vi "TEST - LVOOP Return Class Name.vi"(8 "error in (no error)":errorcluster) -> (0 "error out":errorcluster, 2 "Pass":bool)   [LabVIEW 2020, in "test_openg_array.lvlib"]
uses:
  test_openg_array.lvlib
  LVOOP Data/Class 1/Class 1.lvclass
  source/library/openg_variant.lvlib
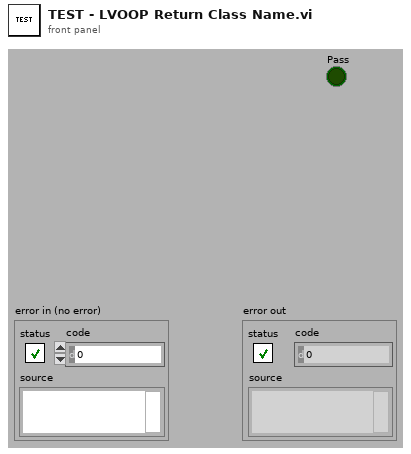
[diagram p1: front panel]
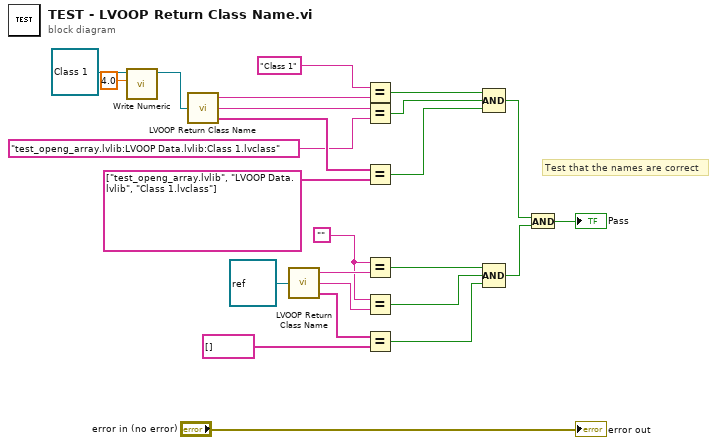
[diagram p0: block diagram]
diagram:
  w19 = ""
  # "Test that the names are correct"
  n1 = call "Write Numeric.vi"("Numeric"=4.0, "Class 1 in"=refnum<class "Class 1.lvclass"> refnum ("Class 1.lvclass")) -> ("Class 1 out"=w2:refnum<class "Class 1.lvclass">)  [unwired: 9 in]
  n2 = call "LVOOP Return Class Name.vi"("Object"=w2) -> ("Class Base Name"=w25:string, "Qualified Name"=w7:string, "Qualified Name Array"=w13:string[])
  n3 = call "LVOOP Return Class Name.vi"("Object"=refnum<class> refnum) -> ("Class Base Name"=w22:string, "Qualified Name"=w20:string, "Qualified Name Array"=w17:string[])
  n4 = Equal?(x="Class 1", y=w25) -> (x = y?=w10:bool)
  n5 = Equal?(x=w7, y="test_openg_array.lvlib:LVOOP Data.lvlib:Class 1.lvclass" ("Fully Qualified Name")) -> (x = y?=w6:bool)
  n6 = Equal?(x=w13, y=string[] ["test_openg_array.lvlib", "LVOOP Data.lvlib", "Class 1.lvclass"] ("Qualified Name Array")) -> (x = y?=w5:bool)
  n7 = Equal?(x=w19, y=w22) -> (x = y?=w14:bool)
  n8 = Equal?(x=w19, y=w20) -> (x = y?=w15:bool)
  n9 = Equal?(x=w17, y=string[] [] ("Qualified Name Array")) -> (x = y?=w16:bool)
  n10 = Compound Arithmetic op=AND(w10, w6, w5) -> (w9:bool)
  n11 = Compound Arithmetic op=AND(w14, w15, w16) -> (w8:bool)
  n12 = And(x=w9, y=w8) -> (x .and. y?=→"Pass":bool)
  "error out" <- "error in (no error)"
